vi "Report Core.vi"(8 "error in":errorcluster, 9 "Received":path, 10 "Approved":path, 11 "Report With LVCompare in":refnum<class "Report With LVCompare.lvclass">) -> (0 "error out":errorcluster, 2 "Worked?":bool, 3 "Report With LVCompare out":refnum<class "Report With LVCompare.lvclass">)   [LabVIEW 2020, in "Approval Tests.lvlib" / "Report With LVCompare.lvclass"]
uses:
  Report With LVCompare.lvclass
  Report With LVCompare.lvclass/Report With LVCompare.ctl
  Approval Tests.lvlib
  OS Strings.ctl
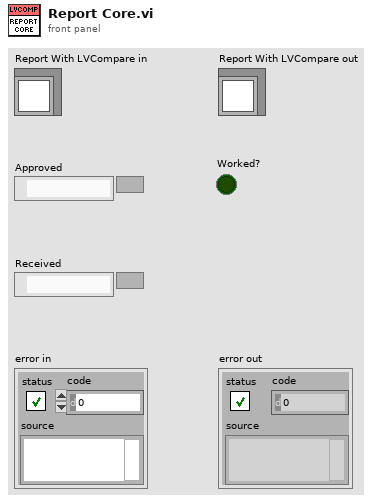
[diagram p1: front panel]
types:
  T1 = typedef "Approval Tests.lvlib/OS Strings.ctl" = cluster{"Windows":string, "Linux":string, "Mac":string}
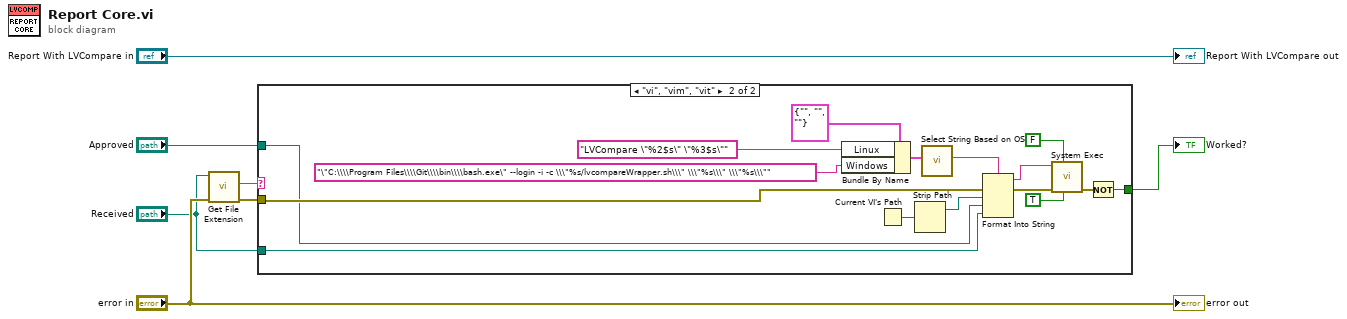
[diagram p0: block diagram]
diagram:
  n1 = call <vilib>:"Get File Extension.vi"("error in (no error)"="error in", "file"="Received") -> ("error out"=w7:errorcluster, "lowercase file extension"=w4:string)  [unwired: 5 in, 3 out]
  n2 = case shown="\"vi\", \"vim\", \"vit\"" w4 {
    tunnel: w7 -> [_ w22]
    tunnel: [_ w20] -> w3
    tunnel: "Approved" -> [_ w15]
    tunnel: "Received" -> [_ w14]
    frame Default {
    }
    frame "vi", "vim", "vit" {
      n3 = Bundle By Name(cluster=T1 {"Windows"="", "Linux"="", "Mac"=""} ("Strings"), "Linux"="LVCompare \"%2$s\" \"%3$s\"", "Windows"="\"C:\\\\Program Files\\\\Git\\\\bin\\\\bash.exe\" --login -i -c \\\"%s/lvcompareWrapper.sh\\\" \\\"%s\\\" \\\"%s\\\"") -> (w10:T1)
      n4 = Current VI's Path() -> (path=w17:path)
      n5 = Strip Path(path=w17) -> (stripped path=w16:path)  [unwired: 1 out]
      n6 = call "Select String Based on OS.vi"("Strings"=w10) -> ("Selection"=w11:string)  [unwired: 10 in]
      n7 = Format Into String(format string=w11, error in=w22, w16, w15, w14) -> (resulting string=w13:string, error out=w21:errorcluster)  [unwired: 1 in]
      n8 = call <vilib>:"System Exec.vi"("run minimized? (F)"=TRUE, "wait until completion? (T)"=FALSE, "error in (no error)"=w21, "command line"=w13) -> ("error out"=w23:errorcluster)  [unwired: 4 in, 3 out]
      n9 = Not(x=w23) -> (.not. x?=w20:bool)
    }
  }
  "Worked?" <- w3
  "error out" <- "error in"
  "Report With LVCompare out" <- "Report With LVCompare in"
